vi "Cluster Literal Probe.vi"() -> ()   [LabVIEW 2026]
doc: "Stage 1: cluster constant literal syntax only. Expected: Named Cluster={1,two,3.5}."
panel:
  out "Named Cluster Out":T1={"Field A"=0, "Field B"="\"\"", "Field C"=0.0}
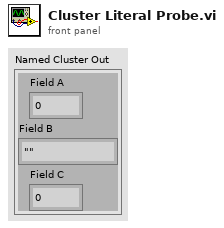
[diagram p1: front panel]
types:
  T1 = cluster{"Field A":i32, "Field B":string, "Field C":dbl}
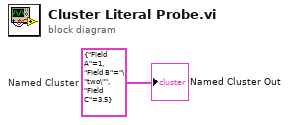
[diagram p0: block diagram]
diagram:
  w1 = T1 {"Field A"=1, "Field B"="\"two\"", "Field C"=3.5}  # Named Cluster
  "Named Cluster Out" <- w1
